vi "Initialize XNET Tree.vi"(4 "Info?":refnum<vi>, 6 "Node Ptr":u64 format="%.0x", 8 "error in":errorcluster, 9 "XNET Cluster":refnum<k21>, 10 "XNET Database":refnum<k21>, 11 "Tree":refnum<vi>) -> (0 "error out":errorcluster, 1 "Parent":string, 2 "XNET Cluster Out":refnum<k21>, 3 "Tree Out":refnum<vi>)   [LabVIEW 2025, in "Protection and Counter Addon System Explorer.lvlib"]
uses:
  Protection and Counter Addon System Explorer.lvlib
  Addon Shared/SubVIs/GUID Lookup.vi
  <resource>/objmgr/xnet.rc
  <vilib>/NI VeriStand/Custom Device API/Custom Device API.lvlib
  Addon Shared/Protection and Counter Addon Shared.lvlib
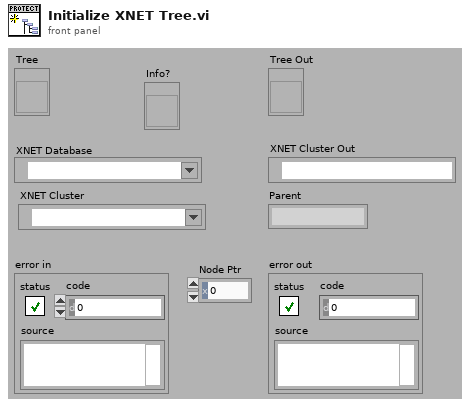
[diagram p1: front panel]
types:
  T1 = typedef "Custom Device API.lvlib/Custom Device Item Info.ctl" = cluster{"Name":string, "Is Channel":bool, "GUID":string, "Is Waveform":bool}
  T2 = typedef "Protection and Counter Addon System Explorer.lvlib/CAN Filter Type.ctl" = enum16{"Cyclic Data", "Event Data", "Cyclic/Event", "All"}
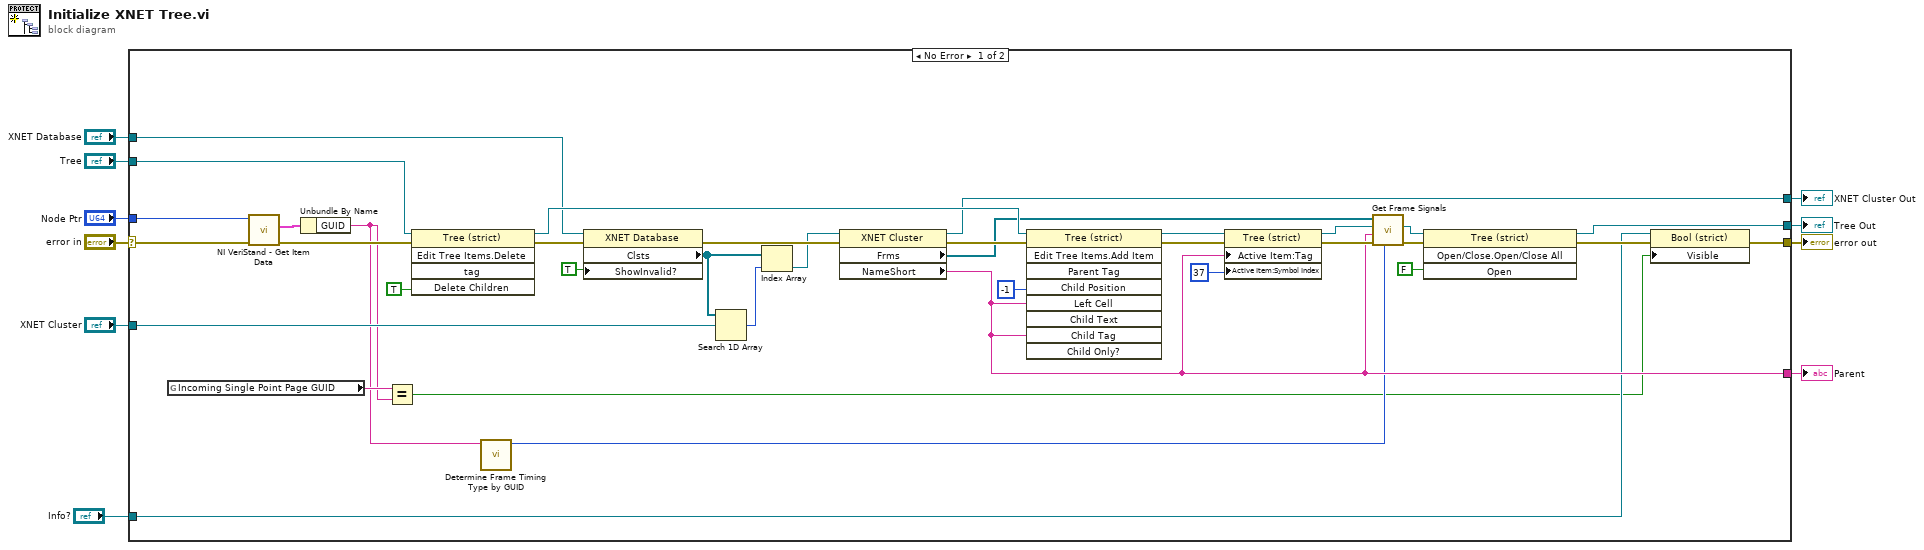
[diagram p0: block diagram]
diagram:
  n1 = case shown="No Error" "error in" {
    selector: "error in" -> [w21 w49]
    tunnel: "Tree" -> [w45 w48]
    tunnel: [w15 w49] -> w9
    tunnel: "XNET Database" -> [w30 _]
    tunnel: [w33 w48] -> w6
    tunnel: [w35 w47] -> w5
    tunnel: "XNET Cluster" -> [w26 w47]
    tunnel: [w22 _] -> w3
    tunnel: "Node Ptr" -> [w19 _]
    tunnel: "Info?" -> [w14 _]
    frame No Error {
      n2 = global read "GUID Lookup.vi" "Incoming Single Point Page GUID"() -> (w12:string)
      n3 = call <vilib>:"NI VeriStand - Get Item Data.vi"("error in (no error)"=w21, "Item Ref in"=w19) -> ("error out"=w20:errorcluster, "Item Info"=w18:T1)  [unwired: 6 in, 2 out]
      n4 = Unbundle By Name(w18) -> ("GUID"=w11:string)
      n5 = Equal?(x=w12, y=w11) -> (x = y?=w13:bool)
      n6 = invoke on="Invoke Node" class="Tree (strict)" method="Edit Tree Items.Delete"(reference=w45, error in=w20, "Delete Children"=TRUE ("Delete Children?")) -> (reference out=w46:refnum<vi>, error out=w28:errorcluster)  [unwired: 2 in, 3 out]
      n7 = call "Determine Frame Timing Type by GUID.vi"("GUID"=w11) -> ("CAN:Frame Type"=w17:T2)  [unwired: 10 in]
      n8 = property class="XNET Database"(reference=w30, error in=w28, "ShowInvalid?"=TRUE ("Show Invalid From Open?")) -> (error out=w27:errorcluster, "Clsts"=w24:refnum<k21>[])  [unwired: 1 out]
      n9 = Search 1D Array(1D array=w24, element=w26) -> (index of element=w25:i32)  [unwired: 1 in]
      n10 = Index Array(array=w24, index=w25) -> (element=w23:refnum<k21>)
      n11 = property class="XNET Cluster"(reference=w23, error in=w27) -> (reference out=w35:refnum<k21>, error out=w37:errorcluster, "Frms"=w36:refnum<k21>[], "NameShort"=w22:string)
      n12 = invoke on="Invoke Node" class="Tree (strict)" method="Edit Tree Items.Add Item"(reference=w46, error in=w37, "Child Position"=-1, "Left Cell"=w22, "Child Tag"=w22) -> (reference out=w40:refnum<vi>, error out=w39:errorcluster)  [unwired: 4 in, 7 out]
      n13 = property class="Tree (strict)"(reference=w40, error in=w39, "Active Item:Tag"=w22, "Active Item:Symbol Index"=37) -> (reference out=w41:refnum<vi>, error out=w42:errorcluster)
      n14 = call "Get Frame Signals.vi"("CAN:Frame Type"=w17, "error in"=w42, "Parent Tag"=w22, "Tree Reference"=w41, "Frms"=w36) -> ("error out"=w32:errorcluster, "Tree Reference Out"=w31:refnum<vi>)  [unwired: 5 in]
      n15 = invoke on="Invoke Node" class="Tree (strict)" method="Open/Close.Open/Close All"(reference=w31, error in=w32, "Open"=FALSE ("Open?")) -> (reference out=w33:refnum<vi>, error out=w16:errorcluster)  [unwired: 1 in, 2 out]
      n16 = property class="Bool (strict)"(reference=w14, error in=w16, "Visible"=w13) -> (error out=w15:errorcluster)  [unwired: 1 out]
    }
    frame Error {
    }
  }
  "error out" <- w9
  "Tree Out" <- w6
  "XNET Cluster Out" <- w5
  "Parent" <- w3
